vi "BIN_find_make_file.vi"(5 "FolderPace":T1, 6 "Max Filesize (bytes)":i64 format="%.0p", 7 "Extension":string, 8 "error in":errorcluster, 9 "TAGs":string[](array[string]), 11 "OpenPattern":path) -> (0 "error out":errorcluster, 2 "New file?":bool, 3 "refnum out":refnum<file>)   [LabVIEW 2020, in "Sgraph_lib_V1.lvlib" / "DBAL-BIN.lvclass"]
doc: "First this method will check if the week number subdirectory exists.\nIf no: then a new folder and historian file will be created with sequence number 001\nIf yes: then the weeknumber folder is searched for the latest file of this resolution layer.\nIf not found: a new file will be created with sequence number 001\nIf found: then the latest sequence of that series is searched.\nIf found and file is small enough: file is opened and reference supplied.\nIf not found or size is too large: New file with sequence number 001 is created."
uses:
  DBAL-BIN.lvclass
  BinFolderPace.ctl
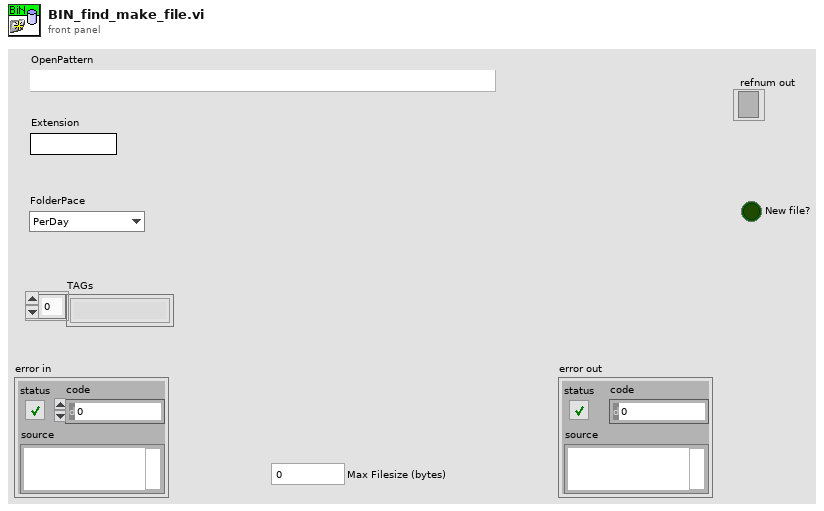
[diagram p1: front panel]
types:
  T1 = typedef "Sgraph_lib_V1.lvlib/DBAL-BIN.lvclass/BinFolderPace.ctl" = enum16{"PerDay", "PerWeek", "PerYear"}
  T2 = enum16{"open", "replace", "create", "open or create", "replace or create", "replace or create with confirmation"}
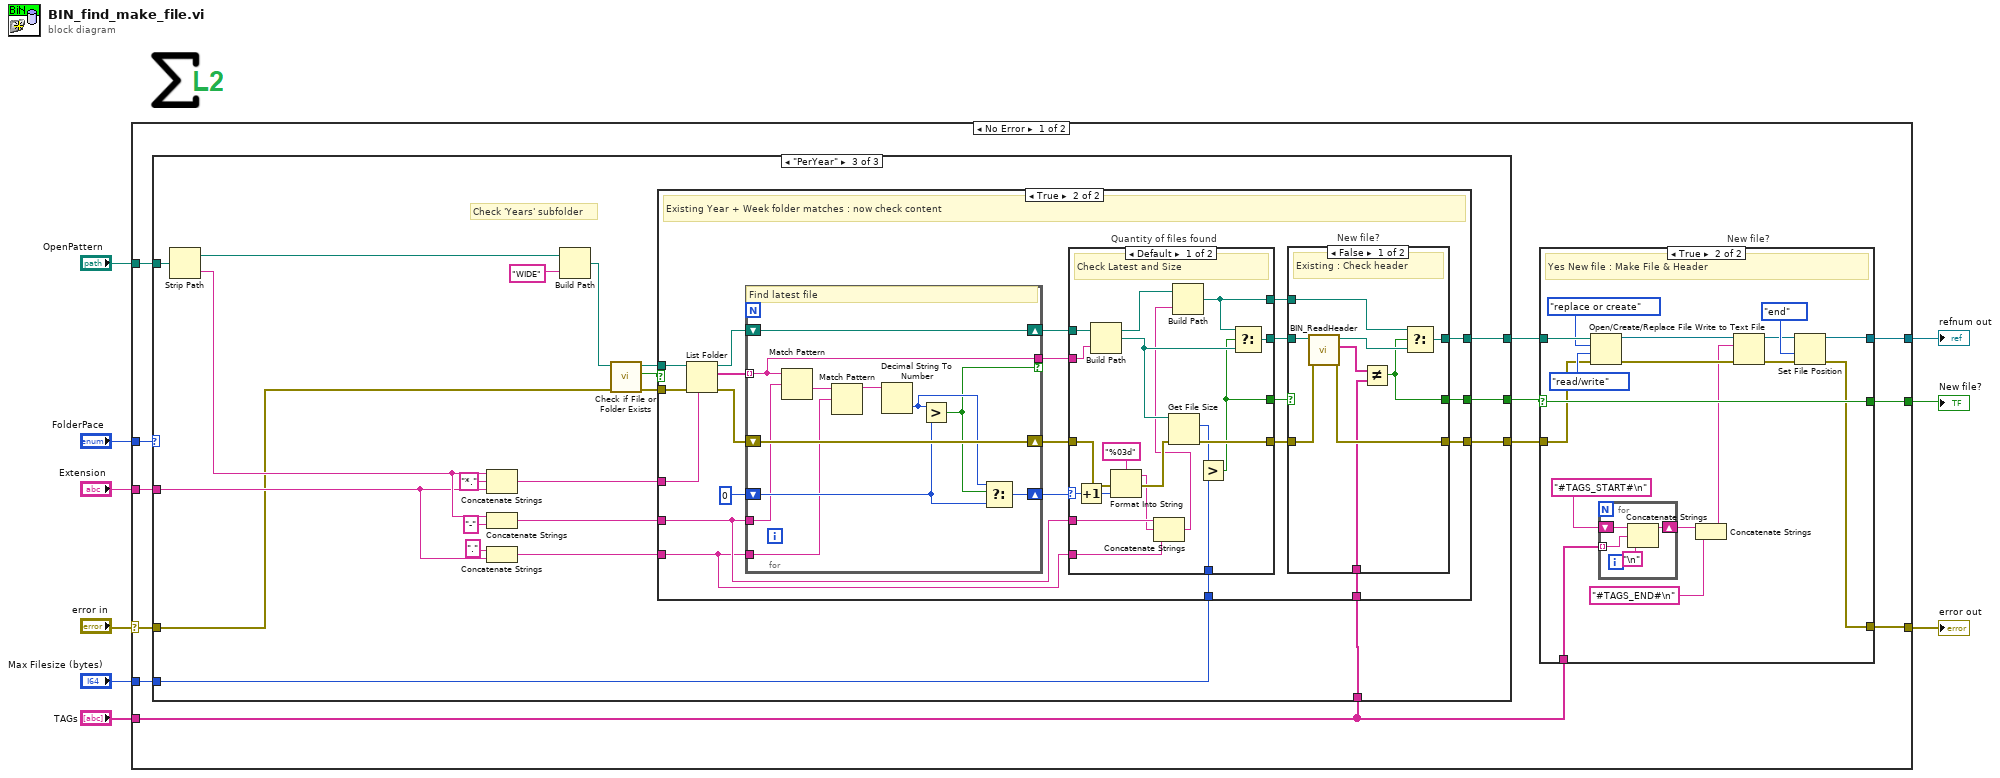
[diagram p0: block diagram]
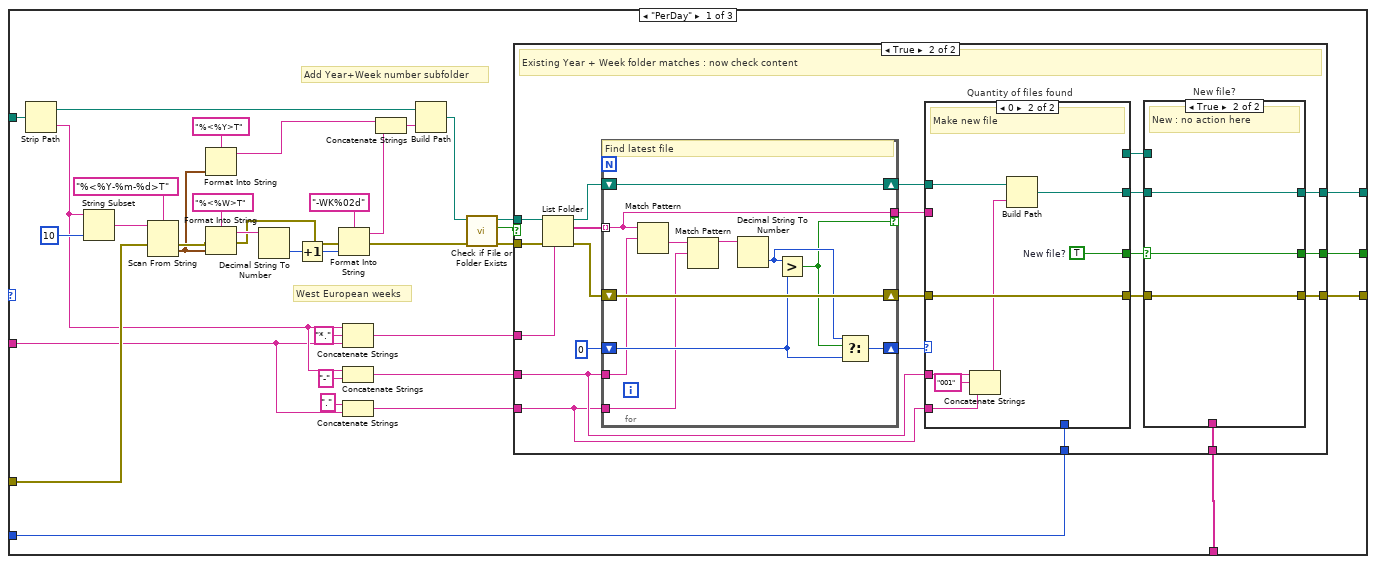
[diagram p2: hidden frame]
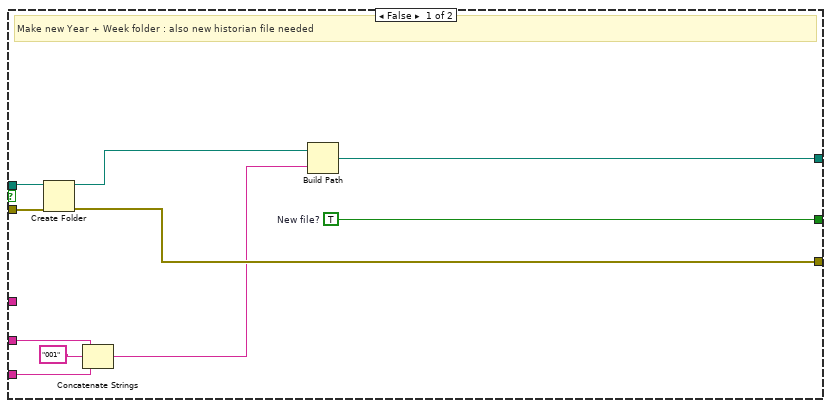
[diagram p3: hidden frame]
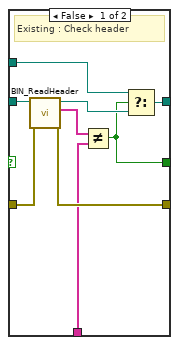
[diagram p4: hidden frame]
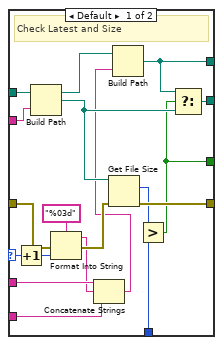
[diagram p5: hidden frame]
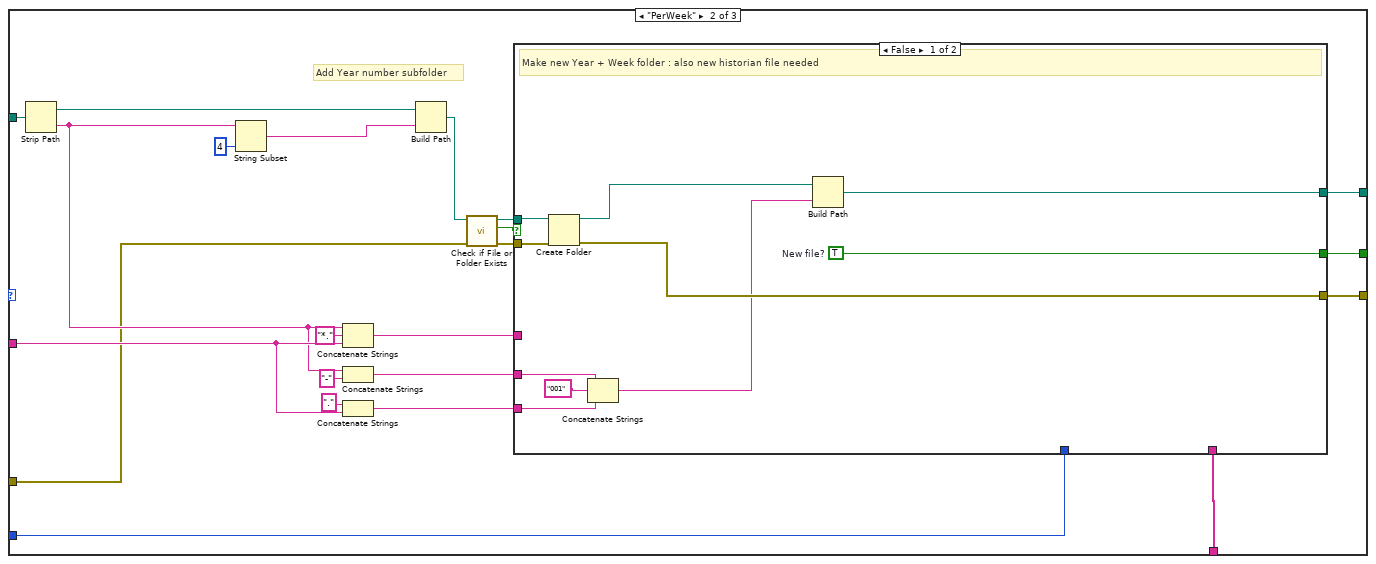
[diagram p6: hidden frame]
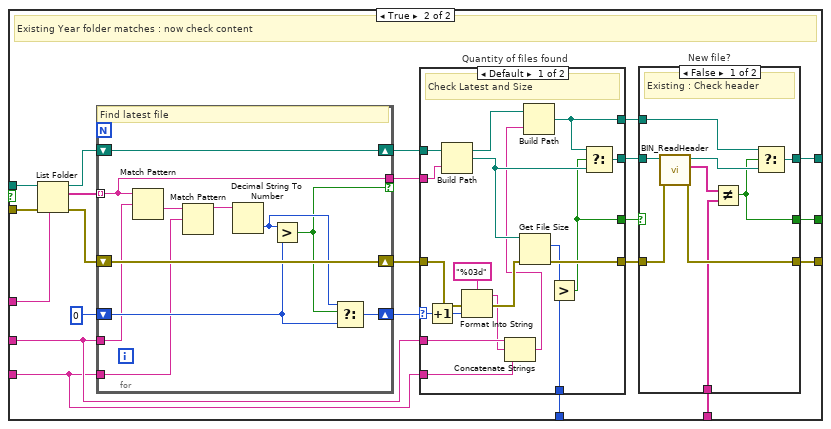
[diagram p7: hidden frame]
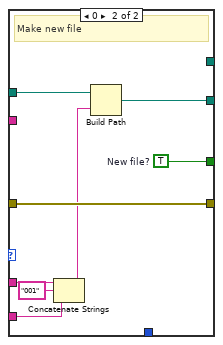
[diagram p9: hidden frame]
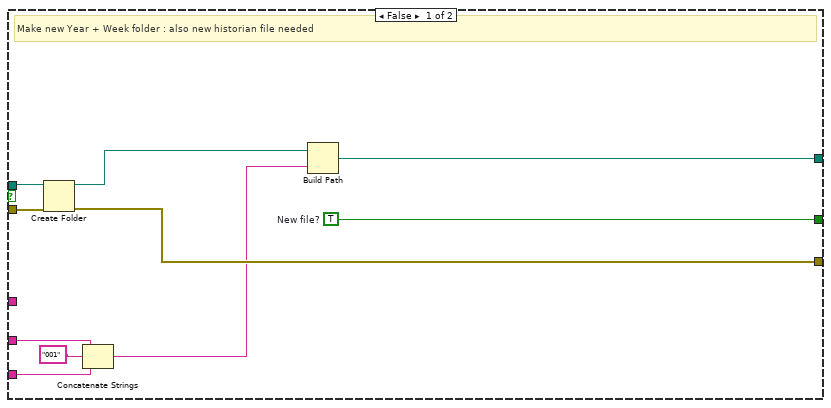
[diagram p10: hidden frame]
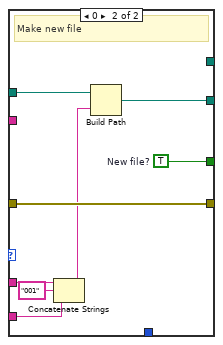
[diagram p12: hidden frame]
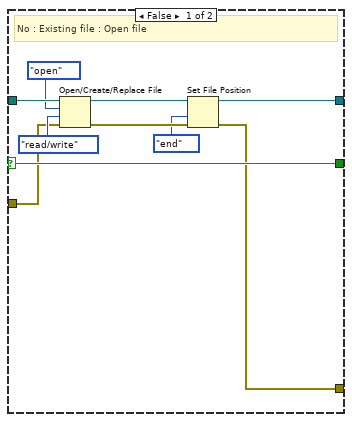
[diagram p13: hidden frame]
diagram:
  n1 = case shown="No Error" "error in" {
    selector: "error in" -> [w20 w375]
    tunnel: [w12 w375] -> w8
    tunnel: "OpenPattern" -> [w21 _]
    tunnel: "Extension" -> [w19 _]
    tunnel: "Max Filesize (bytes)" -> [w18 _]
    tunnel: "TAGs" -> [w14 _]
    tunnel: [w13 _] -> w3
    tunnel: [w11 _] -> w2
    tunnel: "FolderPace" -> [w10 _]
    frame No Error {
      n2 = case shown="\"PerYear\"" w10 {
        tunnel: w21 -> [w57 w160 w262]
        tunnel: w20 -> [w35 w139 w242]
        tunnel: w19 -> [w28 w149 w250]
        tunnel: w18 -> [w26 w147 w248]
        tunnel: [w25 w146 w247] -> w17
        tunnel: [w24 w145 w246] -> w16
        tunnel: [w23 w144 w245] -> w15
        tunnel: w14 -> [w22 w143 w244]
        frame "PerDay" {
          # "West European weeks"
          # "Add Year+Week number subfolder"
          n3 = Strip Path(path=w57) -> (stripped path=w48:path, name=w32:string)
          n4 = String Subset(string=w32, length (rest)=10 ("length (rest)")) -> (substring=w55:string)  [unwired: 1 in]
          n5 = Scan From String(format string="%<%Y-%m-%d>T", input string=w55, error in=w35) -> (error out=w46:errorcluster, output 1=w42:timestamp)  [unwired: 2 in, 2 out]
          n6 = Format Into String(format string="%<%Y>T", w42) -> (resulting string=w39:string)  [unwired: 2 in, 1 out]
          n7 = Format Into String(format string="%<%W>T", error in=w46, w42) -> (resulting string=w52:string, error out=w45:errorcluster)  [unwired: 1 in]
          n8 = Decimal String To Number(string=w52) -> (number=w51:i32)  [unwired: 2 in, 1 out]
          n9 = Increment(x=w51) -> (x+1=w50:i32)
          n10 = Format Into String(format string="-WK%02d", error in=w45, w50) -> (resulting string=w41:string, error out=w44:errorcluster)  [unwired: 1 in]
          n11 = Concatenate Strings(w32, "*." ("string"), w28) -> (w33:string)
          n12 = Concatenate Strings(w32, "-" ("string")) -> (w30:string)
          n13 = Concatenate Strings("." ("string"), w28) -> (w27:string)
          n14 = Concatenate Strings(w39, w41) -> (w40:string)
          n15 = Build Path(base path=w48, name or relative path=w40) -> (appended path=w47:path)
          n16 = call <vilib>:"Check if File or Folder Exists.vi"("error in (no error)"=w44, "path"=w47) -> ("error out"=w36:errorcluster, "file or folder exists?"=w38:bool, "dup path"=w37:path)  [unwired: 7 in]
          n17 = case shown="True" w38 {
            tunnel: w37 -> [w67 w88]
            tunnel: w36 -> [w66 w89]
            tunnel: [w65 w68] -> w25
            tunnel: w33 -> [_ w87]
            tunnel: w30 -> [w60 w78]
            tunnel: w27 -> [w61 w77]
            tunnel: [w64 w69] -> w24
            tunnel: w26 -> [_ w76]
            tunnel: w22 -> [_ w72]
            tunnel: [w58 w70] -> w23
            frame False {
              w64 = TRUE  # New file?
              # "Make new Year + Week folder : also new historian file needed"
              n18 = Create Folder(path (use dialog)=w67, error in=w66) -> (created path=w63:path, error out=w65:errorcluster)  [unwired: 1 in, 1 out]
              n19 = Concatenate Strings(w60, "001" ("string"), w61) -> (w59:string)
              n20 = Build Path(base path=w63, name or relative path=w59) -> (appended path=w58:path)
            }
            frame True {
              # "Existing Year + Week folder matches : now check content"
              n21 = List Folder(path=w88, pattern=w87, error in=w89) -> (path out=w85:path, filenames=w84:string[], error out=w86:errorcluster)  [unwired: 1 in, 1 out]
              n22 = for {
                shift-right: [w136] -> w79
                shift-left: w86 -> [w136]
                shift-right: [w138] -> w81
                shift-left: w85 -> [w138]
                tunnel: w84 -> [w131] mode=indexing
                tunnel: w78 -> [w130]
                tunnel: w77 -> [w129]
                shift-right: [w132] -> w82
                shift-left: 0 -> [w133]
                tunnel: [w131] -> w80 if=w128
                # "Find latest file"
                n23 = Match Pattern(string=w131, regular expression=w130) -> (after substring=w137:string)  [unwired: 1 in, 3 out]
                n24 = Match Pattern(string=w137, regular expression=w129) -> (before substring=w135:string)  [unwired: 1 in, 3 out]
                n25 = Decimal String To Number(string=w135) -> (number=w134:i32)  [unwired: 2 in, 1 out]
                n26 = Greater?(x=w134, y=w133) -> (0:w128:bool)
                n27 = Select(t=w134, s=w128, f=w133) -> (s? t:f=w132:i32)
              }
              n28 = case "Quantity of files found" shown="0" w82 {
                selector: w82 -> [w112 _]
                tunnel: w81 -> [w114 w126]
                tunnel: [w104 w127] -> w75
                tunnel: w80 -> [w119 _]
                tunnel: [w113 w122] -> w74
                tunnel: w78 -> [w107 w125]
                tunnel: w77 -> [w105 w123]
                tunnel: w79 -> [w109 w121]
                tunnel: [w118 w121] -> w73
                tunnel: w76 -> [w116 _]
                tunnel: [w102 _] -> w71
                frame Default {
                  # "Check Latest and Size"
                  n29 = Increment(x=w112) -> (x+1=w111:i32)
                  n30 = Build Path(base path=w114, name or relative path=w119) -> (appended path=w115:path)
                  n31 = Format Into String(format string="%03d", error in=w109, w111) -> (resulting string=w106:string, error out=w108:errorcluster)  [unwired: 1 in]
                  n32 = Concatenate Strings(w107, w106, w105) -> (w103:string)
                  n33 = Get File Size(file=w115, error in=w108) -> (size (in bytes)=w117:i64, 0:w118:errorcluster)  [unwired: 1 out]
                  n34 = Build Path(base path=w114, name or relative path=w103) -> (appended path=w102:path)
                  n35 = Greater?(x=w117, y=w116) -> (0:w104:bool)
                  n36 = Select(t=w102, s=w104, f=w115) -> (s? t:f=w113:path)
                }
                frame 0 {
                  w127 = TRUE  # New file?
                  # "Make new file"
                  n37 = Concatenate Strings(w125, "001" ("string"), w123) -> (w120:string)
                  n38 = Build Path(base path=w126, name or relative path=w120) -> (appended path=w122:path)
                }
              }
              n39 = case "New file?" shown="True" w75 {
                selector: w75 -> [_ w101]
                tunnel: [w90 w101] -> w69
                tunnel: w74 -> [w96 w100]
                tunnel: [w93 w100] -> w70
                tunnel: w73 -> [w98 w99]
                tunnel: [w97 w99] -> w68
                tunnel: w72 -> [w94 _]
                tunnel: w71 -> [w91 _]
                frame False {
                  # "Existing : Check header"
                  n40 = call "BIN_ReadHeader.vi"("error in"=w98, "Path in"=w96) -> ("error out"=w97:errorcluster, "TAGs"=w95:string[], "Path out"=w92:path)  [unwired: 7 in]
                  n41 = Not Equal?(x=w95, y=w94) -> (x != y?=w90:bool)
                  n42 = Select(t=w91, s=w90, f=w92) -> (s? t:f=w93:path)
                }
                frame True {
                  # "New : no action here"
                }
              }
            }
          }
        }
        frame "PerWeek" {
          # "Add Year number subfolder"
          n43 = Strip Path(path=w160) -> (stripped path=w159:path, name=w142:string)
          n44 = String Subset(string=w142, length (rest)=4 ("length (rest)")) -> (substring=w140:string)  [unwired: 1 in]
          n45 = Concatenate Strings(w142, "*." ("string"), w149) -> (w153:string)
          n46 = Concatenate Strings(w142, "-" ("string")) -> (w151:string)
          n47 = Concatenate Strings("." ("string"), w149) -> (w148:string)
          n48 = Build Path(base path=w159, name or relative path=w140) -> (appended path=w158:path)
          n49 = call <vilib>:"Check if File or Folder Exists.vi"("error in (no error)"=w139, "path"=w158) -> ("error out"=w155:errorcluster, "file or folder exists?"=w157:bool, "dup path"=w156:path)  [unwired: 7 in]
          n50 = case shown="False" w157 {
            tunnel: w156 -> [w170 w191]
            tunnel: w155 -> [w169 w192]
            tunnel: [w168 w171] -> w146
            tunnel: w153 -> [_ w190]
            tunnel: w151 -> [w163 w181]
            tunnel: w148 -> [w164 w180]
            tunnel: [w167 w172] -> w145
            tunnel: w147 -> [_ w179]
            tunnel: w143 -> [_ w175]
            tunnel: [w161 w173] -> w144
            frame False {
              w167 = TRUE  # New file?
              # "Make new Year + Week folder : also new historian file needed"
              n51 = Create Folder(path (use dialog)=w170, error in=w169) -> (created path=w166:path, error out=w168:errorcluster)  [unwired: 1 in, 1 out]
              n52 = Concatenate Strings(w163, "001" ("string"), w164) -> (w162:string)
              n53 = Build Path(base path=w166, name or relative path=w162) -> (appended path=w161:path)
            }
            frame True {
              # "Existing Year folder matches : now check content"
              n54 = List Folder(path=w191, pattern=w190, error in=w192) -> (path out=w188:path, filenames=w187:string[], error out=w189:errorcluster)  [unwired: 1 in, 1 out]
              n55 = for {
                shift-right: [w239] -> w182
                shift-left: w189 -> [w239]
                shift-right: [w241] -> w184
                shift-left: w188 -> [w241]
                tunnel: w187 -> [w234] mode=indexing
                tunnel: w181 -> [w233]
                tunnel: w180 -> [w232]
                shift-right: [w235] -> w185
                shift-left: 0 -> [w236]
                tunnel: [w234] -> w183 if=w231
                # "Find latest file"
                n56 = Match Pattern(string=w234, regular expression=w233) -> (after substring=w240:string)  [unwired: 1 in, 3 out]
                n57 = Match Pattern(string=w240, regular expression=w232) -> (before substring=w238:string)  [unwired: 1 in, 3 out]
                n58 = Decimal String To Number(string=w238) -> (number=w237:i32)  [unwired: 2 in, 1 out]
                n59 = Greater?(x=w237, y=w236) -> (0:w231:bool)
                n60 = Select(t=w237, s=w231, f=w236) -> (s? t:f=w235:i32)
              }
              n61 = case "Quantity of files found" shown="Default" w185 {
                selector: w185 -> [w215 _]
                tunnel: w184 -> [w217 w229]
                tunnel: [w207 w230] -> w178
                tunnel: w183 -> [w222 _]
                tunnel: [w216 w225] -> w177
                tunnel: w181 -> [w210 w228]
                tunnel: w180 -> [w208 w226]
                tunnel: w182 -> [w212 w224]
                tunnel: [w221 w224] -> w176
                tunnel: w179 -> [w219 _]
                tunnel: [w205 _] -> w174
                frame Default {
                  # "Check Latest and Size"
                  n62 = Increment(x=w215) -> (x+1=w214:i32)
                  n63 = Build Path(base path=w217, name or relative path=w222) -> (appended path=w218:path)
                  n64 = Format Into String(format string="%03d", error in=w212, w214) -> (resulting string=w209:string, error out=w211:errorcluster)  [unwired: 1 in]
                  n65 = Concatenate Strings(w210, w209, w208) -> (w206:string)
                  n66 = Get File Size(file=w218, error in=w211) -> (size (in bytes)=w220:i64, 0:w221:errorcluster)  [unwired: 1 out]
                  n67 = Build Path(base path=w217, name or relative path=w206) -> (appended path=w205:path)
                  n68 = Greater?(x=w220, y=w219) -> (0:w207:bool)
                  n69 = Select(t=w205, s=w207, f=w218) -> (s? t:f=w216:path)
                }
                frame 0 {
                  w230 = TRUE  # New file?
                  # "Make new file"
                  n70 = Concatenate Strings(w228, "001" ("string"), w226) -> (w223:string)
                  n71 = Build Path(base path=w229, name or relative path=w223) -> (appended path=w225:path)
                }
              }
              n72 = case "New file?" shown="False" w178 {
                selector: w178 -> [_ w204]
                tunnel: [w193 w204] -> w172
                tunnel: w177 -> [w199 w203]
                tunnel: [w196 w203] -> w173
                tunnel: w176 -> [w201 w202]
                tunnel: [w200 w202] -> w171
                tunnel: w175 -> [w197 _]
                tunnel: w174 -> [w194 _]
                frame False {
                  # "Existing : Check header"
                  n73 = call "BIN_ReadHeader.vi"("error in"=w201, "Path in"=w199) -> ("error out"=w200:errorcluster, "TAGs"=w198:string[], "Path out"=w195:path)  [unwired: 7 in]
                  n74 = Not Equal?(x=w198, y=w197) -> (x != y?=w193:bool)
                  n75 = Select(t=w194, s=w193, f=w195) -> (s? t:f=w196:path)
                }
                frame True {
                  # "New : no action here"
                }
              }
            }
          }
        }
        frame "PerYear" {
          # "Check 'Years' subfolder"
          n76 = Strip Path(path=w262) -> (stripped path=w261:path, name=w254:string)
          n77 = Concatenate Strings(w254, "*." ("string"), w250) -> (w255:string)
          n78 = Concatenate Strings(w254, "-" ("string")) -> (w252:string)
          n79 = Concatenate Strings("." ("string"), w250) -> (w249:string)
          n80 = Build Path(base path=w261, name or relative path="WIDE" ("format string")) -> (appended path=w260:path)
          n81 = call <vilib>:"Check if File or Folder Exists.vi"("error in (no error)"=w242, "path"=w260) -> ("error out"=w257:errorcluster, "file or folder exists?"=w259:bool, "dup path"=w258:path)  [unwired: 7 in]
          n82 = case shown="True" w259 {
            tunnel: w258 -> [w272 w293]
            tunnel: w257 -> [w271 w294]
            tunnel: [w270 w273] -> w247
            tunnel: w255 -> [_ w292]
            tunnel: w252 -> [w265 w283]
            tunnel: w249 -> [w266 w282]
            tunnel: [w269 w274] -> w246
            tunnel: w248 -> [_ w281]
            tunnel: w244 -> [_ w277]
            tunnel: [w263 w275] -> w245
            frame False {
              w269 = TRUE  # New file?
              # "Make new Year + Week folder : also new historian file needed"
              n83 = Create Folder(path (use dialog)=w272, error in=w271) -> (created path=w268:path, error out=w270:errorcluster)  [unwired: 1 in, 1 out]
              n84 = Concatenate Strings(w265, "001" ("string"), w266) -> (w264:string)
              n85 = Build Path(base path=w268, name or relative path=w264) -> (appended path=w263:path)
            }
            frame True {
              # "Existing Year + Week folder matches : now check content"
              n86 = List Folder(path=w293, pattern=w292, error in=w294) -> (path out=w290:path, filenames=w289:string[], error out=w291:errorcluster)  [unwired: 1 in, 1 out]
              n87 = for {
                shift-right: [w341] -> w284
                shift-left: w291 -> [w341]
                shift-right: [w343] -> w286
                shift-left: w290 -> [w343]
                tunnel: w289 -> [w336] mode=indexing
                tunnel: w283 -> [w335]
                tunnel: w282 -> [w334]
                shift-right: [w337] -> w287
                shift-left: 0 -> [w338]
                tunnel: [w336] -> w285 if=w333
                # "Find latest file"
                n88 = Match Pattern(string=w336, regular expression=w335) -> (after substring=w342:string)  [unwired: 1 in, 3 out]
                n89 = Match Pattern(string=w342, regular expression=w334) -> (before substring=w340:string)  [unwired: 1 in, 3 out]
                n90 = Decimal String To Number(string=w340) -> (number=w339:i32)  [unwired: 2 in, 1 out]
                n91 = Greater?(x=w339, y=w338) -> (0:w333:bool)
                n92 = Select(t=w339, s=w333, f=w338) -> (s? t:f=w337:i32)
              }
              n93 = case "Quantity of files found" shown="Default" w287 {
                selector: w287 -> [w317 _]
                tunnel: w286 -> [w319 w331]
                tunnel: [w309 w332] -> w280
                tunnel: w285 -> [w324 _]
                tunnel: [w318 w327] -> w279
                tunnel: w283 -> [w312 w330]
                tunnel: w282 -> [w310 w328]
                tunnel: w284 -> [w314 w326]
                tunnel: [w323 w326] -> w278
                tunnel: w281 -> [w321 _]
                tunnel: [w307 _] -> w276
                frame Default {
                  # "Check Latest and Size"
                  n94 = Increment(x=w317) -> (x+1=w316:i32)
                  n95 = Build Path(base path=w319, name or relative path=w324) -> (appended path=w320:path)
                  n96 = Format Into String(format string="%03d", error in=w314, w316) -> (resulting string=w311:string, error out=w313:errorcluster)  [unwired: 1 in]
                  n97 = Concatenate Strings(w312, w311, w310) -> (w308:string)
                  n98 = Get File Size(file=w320, error in=w313) -> (size (in bytes)=w322:i64, 0:w323:errorcluster)  [unwired: 1 out]
                  n99 = Build Path(base path=w319, name or relative path=w308) -> (appended path=w307:path)
                  n100 = Greater?(x=w322, y=w321) -> (0:w309:bool)
                  n101 = Select(t=w307, s=w309, f=w320) -> (s? t:f=w318:path)
                }
                frame 0 {
                  w332 = TRUE  # New file?
                  # "Make new file"
                  n102 = Concatenate Strings(w330, "001" ("string"), w328) -> (w325:string)
                  n103 = Build Path(base path=w331, name or relative path=w325) -> (appended path=w327:path)
                }
              }
              n104 = case "New file?" shown="False" w280 {
                selector: w280 -> [_ w306]
                tunnel: [w295 w306] -> w274
                tunnel: w279 -> [w301 w305]
                tunnel: [w298 w305] -> w275
                tunnel: w278 -> [w303 w304]
                tunnel: [w302 w304] -> w273
                tunnel: w277 -> [w299 _]
                tunnel: w276 -> [w296 _]
                frame False {
                  # "Existing : Check header"
                  n105 = call "BIN_ReadHeader.vi"("error in"=w303, "Path in"=w301) -> ("error out"=w302:errorcluster, "TAGs"=w300:string[], "Path out"=w297:path)  [unwired: 7 in]
                  n106 = Not Equal?(x=w300, y=w299) -> (x != y?=w295:bool)
                  n107 = Select(t=w296, s=w295, f=w297) -> (s? t:f=w298:path)
                }
                frame True {
                  # "New : no action here"
                }
              }
            }
          }
        }
      }
      n108 = case "New file?" shown="True" w16 {
        selector: w16 -> [w353 w370]
        tunnel: [w353 w370] -> w13
        tunnel: w15 -> [w352 w369]
        tunnel: [w348 w354] -> w11
        tunnel: w17 -> [w346 w366]
        tunnel: [w345 w357] -> w12
        tunnel: w14 -> [_ w365]
        frame False {
          # "No : Existing file : Open file"
          n109 = Open/Create/Replace File(file path (use dialog)=w352, error in=w346, operation (0:open)=T2."open", access (0:read/write)=enum16{"read/write", "read-only", "write-only"}."read/write") -> (refnum out=w349:refnum<file>, error out=w347:errorcluster)  [unwired: 2 in, 1 out]
          n110 = Set File Position(refnum=w349, from (0:start)=enum16{"start", "end", "current"}."end", error in=w347) -> (refnum out=w348:refnum<file>, error out=w345:errorcluster)  [unwired: 1 in]
        }
        frame True {
          # "Yes New file : Make File & Header"
          n111 = Open/Create/Replace File(file path (use dialog)=w369, error in=w366, operation (0:open)=T2."replace or create", access (0:read/write)=enum16{"read/write", "read-only", "write-only"}."read/write") -> (refnum out=w360:refnum<file>, error out=w358:errorcluster)  [unwired: 2 in, 1 out]
          n112 = for {
            tunnel: w365 -> [w373] mode=indexing
            shift-right: [w372] -> w363
            shift-left: "#TAGS_START#\n" -> [w374]
            n113 = Concatenate Strings(w374, w373, "\n") -> (w372:string)
          }
          n114 = Concatenate Strings(w363, "#TAGS_END#\n") -> (w356:string)
          n115 = Write to Text File(file (use dialog)=w360, text=w356, error in=w358) -> (refnum out=w355:refnum<file>, error out=w359:errorcluster)  [unwired: 1 in, 1 out]
          n116 = Set File Position(refnum=w355, from (0:start)=enum16{"start", "end", "current"}."end", error in=w359) -> (refnum out=w354:refnum<file>, error out=w357:errorcluster)  [unwired: 1 in]
        }
      }
    }
    frame Error {
    }
  }
  "error out" <- w8
  "New file?" <- w3
  "refnum out" <- w2
